vi "TCP Server Get Process VI Paths.vi"() -> (0 "Processes":string[](array[string]))   [LabVIEW 2020, in "JKI TCP Server.lvclass"]
uses:
  JKI TCP Server.lvclass
panel:
  in  "Case Constant\n(See Context Help)":bool
  # "Copyright © 2004-2008 JKI. All rights reserved.\n\nAuthor: Jim Kring [jim.kring@jameskring.com]\n\nThis library is provided \"AS IS\" ,WITHOUT WARRANTIES OR \nCONDITIONS OF ANY KIND, either express or implied.\n\nJames Kring, Inc. -- http://www.jameskring.com"
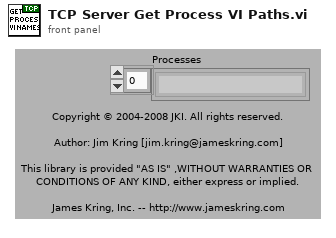
[diagram p1: front panel]
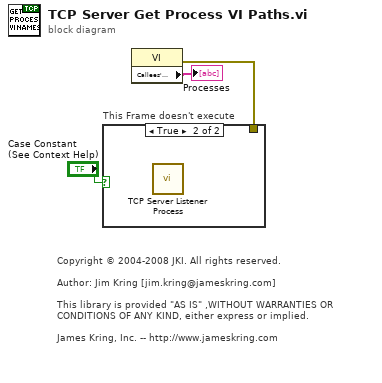
[diagram p0: block diagram]
diagram:
  # "Copyright © 2004-2008 JKI. All rights reserved.\n\nAuthor: Jim Kring [jim.kring@jameskring.com]\n\nThis library is provided \"AS IS\" ,WITHOUT WARRANTIES OR \nCONDITIONS OF ANY KIND, either express or implied.\n\nJames Kring, Inc. -- http://www.jameskring.com"
  n1 = property class="VI"() -> (error out=w1:errorcluster, "Callees' Names"=→"Processes":string[])  [unwired: 2 in, 1 out]
  n2 = case "This Frame doesn't execute" shown="True" "Case Constant\n(See Context Help)" {
    tunnel: w1 -> [_ _]
    frame False {
    }
    frame True {
      n3 = call "TCP Server Listener Process.vi"() -> ()  [unwired: 1 in]
    }
  }
